vi "Set Tab Page.vi"(8 "error in (no error)":errorcluster, 10 "PageOfTab":string, 11 "VI in":refnum<vi>) -> (0 "error out":errorcluster, 3 "VI out":refnum<vi>)   [LabVIEW 2019, in "Language Editor.lvlib"]
doc: "- - -\nCopyright (c) 2026, Merecs Engineering GmbH"
uses:
  Language Editor.lvlib
panel:
  # "Connector Pane"
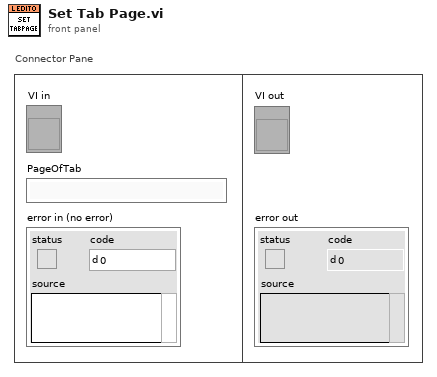
[diagram p1: front panel]
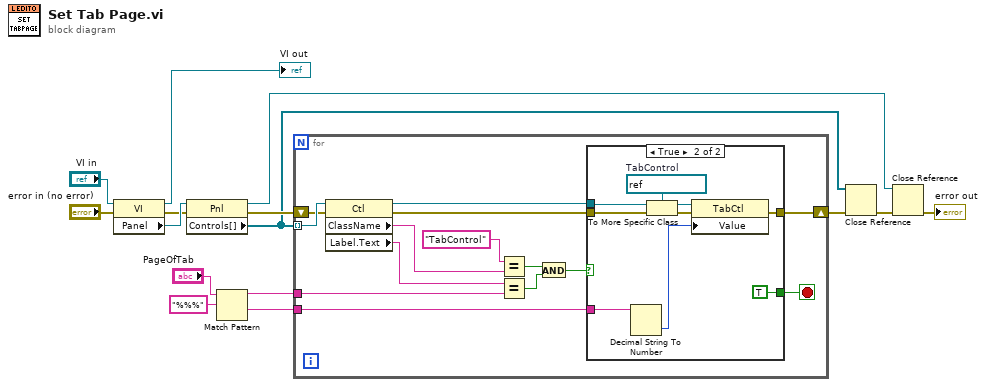
[diagram p0: block diagram]
diagram:
  n1 = property class="VI"(reference="VI in", error in="error in (no error)") -> (reference out=→"VI out":refnum<vi>, error out=w10:errorcluster, "Panel"=w15:refnum<vi>)
  n2 = property class="Pnl"(reference=w15, error in=w10) -> (reference out=w5:refnum<vi>, error out=w9:errorcluster, "Controls[]"=w6:refnum<vi>[])
  n3 = Match Pattern(string="PageOfTab", regular expression="%%%" ("string")) -> (before substring=w8:string, after substring=w7:string)  [unwired: 1 in, 2 out]
  n4 = for {
    tunnel: w6 -> [w29] mode=indexing
    shift-right: [w17] -> w4
    shift-left: w9 -> [w28]
    tunnel: w8 -> [w24]
    tunnel: w7 -> [w19]
    stop <- w16 stop-if-true
    n5 = property class="Ctl"(reference=w29, error in=w28) -> (reference out=w21:refnum<vi>, error out=w18:errorcluster, "ClassName"=w27:string, "Label.Text"=w25:string)
    n6 = Equal?(x="TabControl", y=w27) -> (x = y?=w23:bool)
    n7 = Equal?(x=w25, y=w24) -> (x = y?=w22:bool)
    n8 = And(x=w23, y=w22) -> (x .and. y?=w20:bool)
    n9 = case shown="True" w20 {
      tunnel: w21 -> [_ w37]
      tunnel: w19 -> [_ w32]
      tunnel: w18 -> [w30 w39]
      tunnel: [w30 w38] -> w17
      tunnel: [_ TRUE] -> w16
      frame False {
      }
      frame True {
        w36 = refnum<vi> refnum  # TabControl
        n10 = Decimal String To Number(string=w32) -> (number=w31:i32)  [unwired: 2 in, 1 out]
        n11 = To More Specific Class(target class=w36, reference=w37, error in=w39) -> (specific class reference=w35:refnum<vi>, error out=w34:errorcluster)
        n12 = property class="TabCtl"(reference=w35, error in=w34, "Value"=w31) -> (error out=w38:errorcluster)  [unwired: 1 out]
      }
    }
  }
  n13 = Close Reference(reference=w6, error in (no error)=w4) -> (error out=w3:errorcluster)
  n14 = Close Reference(reference=w5, error in (no error)=w3) -> (error out=→"error out":errorcluster)
